vi "Conv_POSE2D_SI_Eng.vi"(11 "Err Pose in SI":T1 {"ROTATION"."SIN" format="%13.4f"; "ROTATION"."COS" format="%13.4f"; "ROTATION"."VALUE" format="%13.4f"; "TRANSLATION"."Y" format="%14.3f"; "TRANSLATION"."X" format="%14.3f"}) -> (3 "Err Pose out ENG":T1 {"ROTATION"."SIN" format="%13.4f"; "ROTATION"."COS" format="%13.4f"; "ROTATION"."VALUE" format="%13.4f"; "TRANSLATION"."Y" format="%14.3f"; "TRANSLATION"."X" format="%14.3f"})   [LabVIEW 2019, in "Trajectory_Library.lvlib"]
doc: "Convert POSE from Meters, Radians to Feet, Radians. (Rotation2d is always expressed as radians.) (This is really only for external use. All the internal routines use meters and radians.)"
uses:
  Trajectory_Library.lvlib
  TypeDef/POSE2D.ctl
  TypeDef/TRANSLATION2D.ctl
  TypeDef/ROTATION2D.ctl
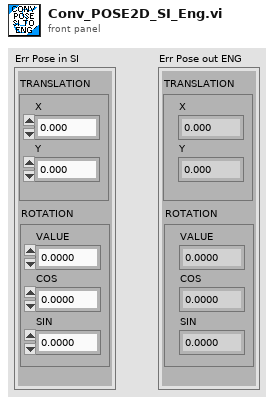
[diagram p1: front panel]
types:
  T1 = typedef "Trajectory_Library.lvlib/POSE2D.ctl" = cluster{"TRANSLATION":T2, "ROTATION":T3}
  T2 = typedef "Trajectory_Library.lvlib/TRANSLATION2D.ctl" = cluster{"X":dbl, "Y":dbl}
  T3 = typedef "Trajectory_Library.lvlib/ROTATION2D.ctl" = cluster{"VALUE":dbl, "COS":dbl, "SIN":dbl}
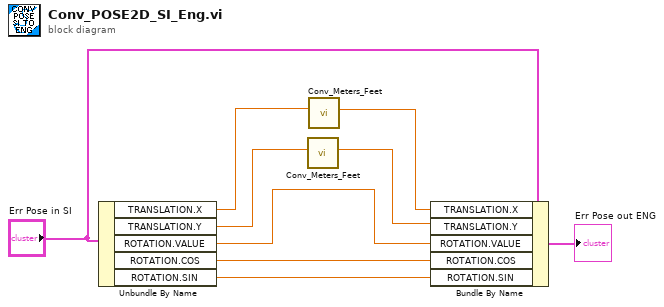
[diagram p0: block diagram]
diagram:
  n1 = Unbundle By Name("Err Pose in SI") -> ("TRANSLATION.X"=w7:dbl, "TRANSLATION.Y"=w5:dbl, "ROTATION.VALUE"=w1:dbl, "ROTATION.COS"=w3:dbl, "ROTATION.SIN"=w2:dbl)
  n2 = call "Conv_Meters_Feet.vi"("Meters"=w5) -> ("Feet"=w4:dbl)  [unwired: 10 in]
  n3 = call "Conv_Meters_Feet.vi"("Meters"=w7) -> ("Feet"=w6:dbl)  [unwired: 10 in]
  n4 = Bundle By Name(cluster="Err Pose in SI", "TRANSLATION.X"=w6, "TRANSLATION.Y"=w4, "ROTATION.VALUE"=w1, "ROTATION.COS"=w3, "ROTATION.SIN"=w2) -> (→"Err Pose out ENG":T1)
